vi "ExecutableInstance.vi"(8 "error in (no error)":errorcluster) -> (0 "error out":errorcluster)   [LabVIEW 2016, in "DronaTest.lvlib"]
uses:
  DronaTest.lvlib
  <vilib>/addons/_JKI Toolkits/Caraya/classes/Assert/Assert Not Error.vi
  <vilib>/addons/_JKI Toolkits/Caraya/classes/Assert/Assert.lvclass
  <vilib>/addons/_JKI Toolkits/Caraya/classes/Test/Test.lvclass
  <vilib>/Utility/LVLibp/NI_PackedLibraryUtility.lvlib
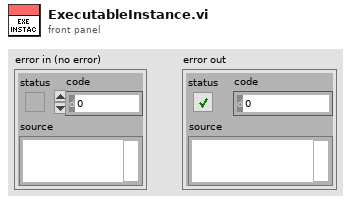
[diagram p1: front panel]
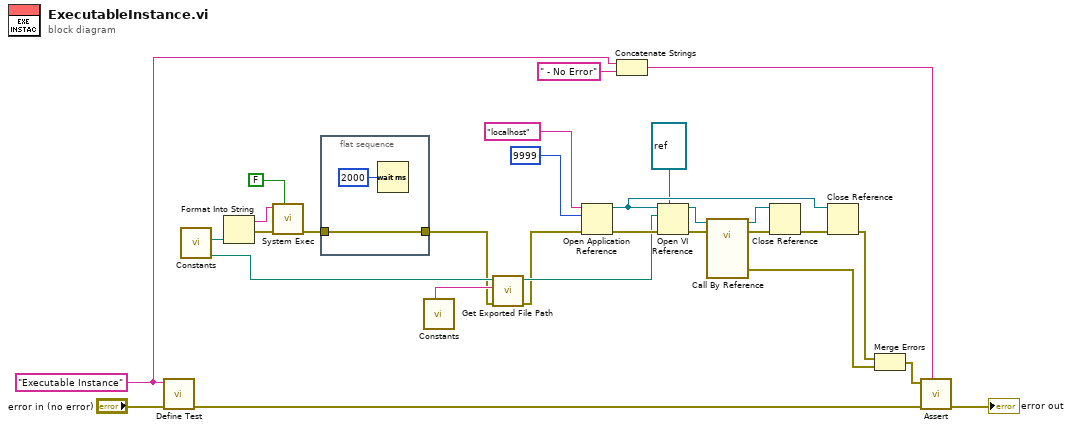
[diagram p0: block diagram]
diagram:
  w18 = "Executable Instance" ("Label (VI Title)")
  n1 = call <vilib>:"Define Test.vi"("error in (no error)"="error in (no error)", "Label (VI Title)"=w18) -> ("error out"=w26:errorcluster)  [unwired: 9 in]
  n2 = call "Constants.vi"() -> ("TestPPL Path"=w5:path, "HelperExecutable path"=w19:path)  [unwired: 5 in, 5 out]
  n3 = Format Into String(w19) -> (resulting string=w22:string, error out=w23:errorcluster)  [unwired: 3 in]
  n4 = call <vilib>:"System Exec.vi"("wait until completion? (T)"=FALSE, "error in (no error)"=w23, "command line"=w22) -> ("error out"=w20:errorcluster)  [unwired: 5 in, 3 out]
  n5 = flat-sequence {
    tunnel: [w31] -> w1
    tunnel: w20 -> [w31]
    frame #0 {
      n6 = Wait (ms)(milliseconds to wait=u32 2000) -> ()  [unwired: 1 out]
    }
  }
  n7 = call "Constants.vi"() -> ("PPL Name"=w3:string)  [unwired: 5 in, 6 out]
  n8 = call <vilib>:"Get Exported File Path.vi"("error in (no error)"=w1, "qualified name"=w3, "packed library path"=w5) -> ("error out"=w2:errorcluster, "path"=w4:path)  [unwired: 7 in]
  n9 = Open Application Reference(8:w2, 10:u16 9999 ("Port(0:Ignored)"), 11:"localhost" ("Project Name (\"\": ThisApplication)")) -> (0:w15:errorcluster, 3:w14:refnum<vi>)  [unwired: 1 in]
  n10 = Concatenate Strings(w18, " - No Error" ("Label (VI Title)")) -> (w24:string)
  n11 = Open VI Reference(type specifier VI Refnum (for type only)=refnum<vi> refnum, application reference (local)=w14, vi path=w4, error in (no error)=w15) -> (vi reference=w6:refnum<vi>, error out=w9:errorcluster)  [unwired: 2 in]
  n12 = call-by-ref "?"(reference=w6, error in=w9) -> (reference out=w7:refnum<vi>, error out=w8:errorcluster, 15:"error out"=w11:errorcluster)  [unwired: 15 in]
  n13 = Close Reference(reference=w7, error in (no error)=w8) -> (error out=w10:errorcluster)
  n14 = Close Reference(reference=w14, error in (no error)=w10) -> (error out=w12:errorcluster)
  n15 = Merge Errors(w12, w11) -> (w29:errorcluster)
  n16 = call-poly <vilib>:"Assert.vi"("Label"=w24, "error in (no error)"=w26, "Not Error?"=w29) -> ("error out"=→"error out":errorcluster)  [unwired: 8 in]
